vi "FuncVI_Sub - VI - Set VI control value.vi"(6 "type":T1=enum."Unknown data type", 7 "control name":string, 8 "error in":errorcluster, 9 "str":string, 10 "dbl":dbl, 11 "VI Ref":refnum<vi>) -> (0 "error out":errorcluster, 3 "dup VI Ref":refnum<vi>)   [LabVIEW 2021]
doc: "::: CalcExpress Toolkit :::\nCopyright (c) 2000-2026 Konstantin Shifershteyn. All rights reserved."
uses:
  cetypes.llb/CalcExpress Data Type.ctl
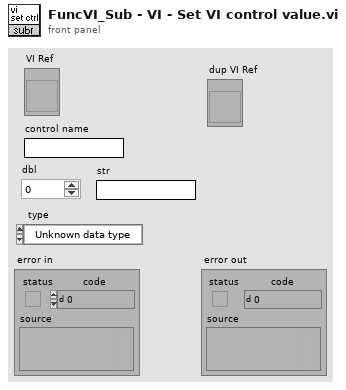
[diagram p1: front panel]
types:
  T1 = typedef "CalcExpress Data Type.ctl" = enum32{"String", "DBL Number", "identifier", "1D Array of DBL", "2D Array of DBL", "CDB Number", "1D Array of CDB", "2D Array of CDB", "1D Array of String", "2D Array of String", "Unknown data type"}
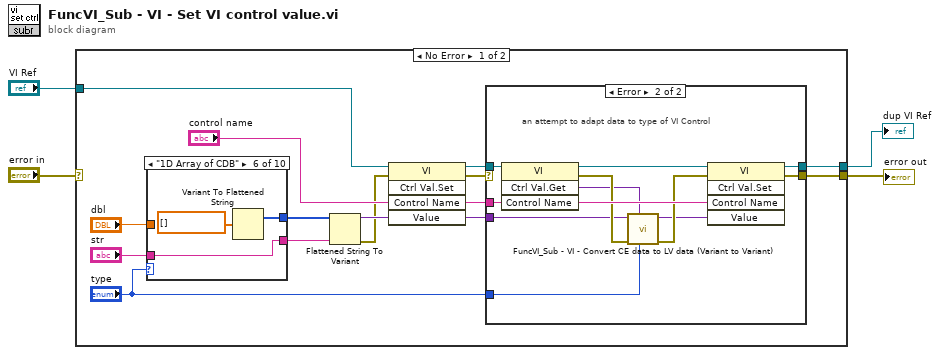
[diagram p0: block diagram]
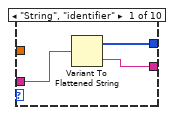
[diagram p3: hidden frame]
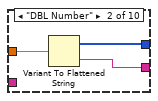
[diagram p4: hidden frame]
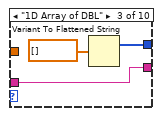
[diagram p5: hidden frame]
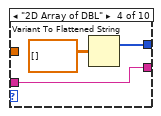
[diagram p6: hidden frame]
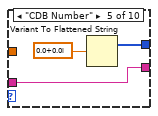
[diagram p7: hidden frame]
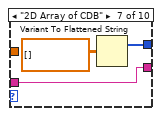
[diagram p8: hidden frame]
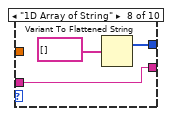
[diagram p9: hidden frame]
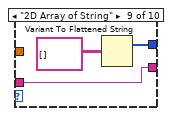
[diagram p10: hidden frame]
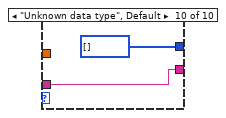
[diagram p11: hidden frame]
diagram:
  n1 = case shown="No Error" "error in" {
    selector: "error in" -> [_ w60]
    tunnel: "VI Ref" -> [w9 w61]
    tunnel: [w13 w60] -> w3
    tunnel: [w12 w61] -> w2
    frame No Error {
      n2 = case shown="\"1D Array of CDB\"" "type" {
        tunnel: [w32 w35 w39 w42 w45 w48 w51 w54 w57 i16[] [] ("type string")] -> w10
        tunnel: [w31 w34 w38 w41 w44 w47 w50 w53 w56 w59] -> w8
        tunnel: "dbl" -> [_ w36 _ _ _ _ _ _ _ _]
        tunnel: "str" -> [w33 _ w38 w41 w44 w47 w50 w53 w56 w59]
        frame "String", "identifier" {
          n3 = Variant To Flattened String(Variant=w33) -> (data string=w31:string, 1:w32:i16[])
        }
        frame "DBL Number" {
          n4 = Variant To Flattened String(Variant=w36) -> (data string=w34:string, 1:w35:i16[])
        }
        frame "1D Array of DBL" {
          n5 = Variant To Flattened String(Variant=dbl[] []) -> (1:w39:i16[])  [unwired: 1 out]
        }
        frame "2D Array of DBL" {
          n6 = Variant To Flattened String(Variant=dbl[][] []) -> (1:w42:i16[])  [unwired: 1 out]
        }
        frame "CDB Number" {
          n7 = Variant To Flattened String(Variant=cdb 0.0+0.0i) -> (1:w45:i16[])  [unwired: 1 out]
        }
        frame "1D Array of CDB" {
          n8 = Variant To Flattened String(Variant=cdb[] []) -> (1:w48:i16[])  [unwired: 1 out]
        }
        frame "2D Array of CDB" {
          n9 = Variant To Flattened String(Variant=cdb[][] []) -> (1:w51:i16[])  [unwired: 1 out]
        }
        frame "1D Array of String" {
          n10 = Variant To Flattened String(Variant=string[] []) -> (1:w54:i16[])  [unwired: 1 out]
        }
        frame "2D Array of String" {
          n11 = Variant To Flattened String(Variant=string[][] []) -> (1:w57:i16[])  [unwired: 1 out]
        }
        frame "Unknown data type", Default {
        }
      }
      n12 = Flattened String To Variant(6:w8, 7:w10) -> (0:w5:errorcluster, 3:w6:variant)  [unwired: 1 in]
      n13 = invoke class="VI" method="Ctrl Val.Set"(reference=w9, error in=w5, "Control Name"="control name", "Value"=w6) -> (reference out=w15:refnum<vi>, error out=w11:errorcluster)  [unwired: 1 in, 3 out]
      n14 = case shown="Error" w11 {
        selector: w11 -> [w18 _]
        tunnel: w15 -> [w19 w30]
        tunnel: "control name" -> [_ w29]
        tunnel: "type" -> [_ w23]
        tunnel: [w19 w28] -> w12
        tunnel: [w18 w26] -> w13
        tunnel: w6 -> [_ w21]
        frame No Error {
        }
        frame Error {
          # "an attempt to adapt data to type of VI Control"
          n15 = invoke class="VI" method="Ctrl Val.Get"(reference=w30, "Control Name"=w29) -> (reference out=w27:refnum<vi>, error out=w25:errorcluster, "Get Control Value Variant"=w20:variant)  [unwired: 2 in, 1 out]
          n16 = call "FuncVI_Sub - VI - Convert CE data to LV data (Variant to Variant).vi"("CE data type"=w23, "LV data (typedef)"=w20, "error in"=w25, "CE data"=w21) -> ("error out"=w24:errorcluster, "LV data out"=w22:variant)  [unwired: 6 in]
          n17 = invoke class="VI" method="Ctrl Val.Set"(reference=w27, error in=w24, "Control Name"=w29, "Value"=w22) -> (reference out=w28:refnum<vi>, error out=w26:errorcluster)  [unwired: 1 in, 3 out]
        }
      }
    }
    frame Error {
    }
  }
  "dup VI Ref" <- w2
  "error out" <- w3
